vi "RemoteVI Complex Fixture.vi"() -> ()   [LabVIEW 2020]
doc: "This example demonstrates the use of splitter bars to divide the front panel into multiple panes. Each pane can be set up to behave differently depending on the desired function of each pane. In this example the graphical display contained in the lower right pane has the ability to resize with the pane."
uses:
  source/RemoteVI.lvlib
panel:
  in  "Nav":string(tree)="tag_item1"
  out "error out":errorcluster
  in  "Inspector":bool
  in  "Stop":bool
  in  "Steps":cluster{"Name":string, "Value":dbl, "On":bool}[](array[cluster])
  in  "Results":string[][](table)
  in  "Log Path":path
  out "Status":string
  in  "View":i32(ring) items=["View A", "View B"]
  in  "Settings":enum32{"Acquisition", "Display", "Viewer"}(tab)
  in  "Channel":T1
  in  "Rate":dbl(slide)=154517.79084245834 scale=1.0..205410.22592152198 scale format="%#_6p"
  in  "Level":dbl(knob)=22413.793103448275 scale=1.0..100000.0 scale format="%#_6p"
  in  "Data File":path
  out "Scope":dbl[][](graph)
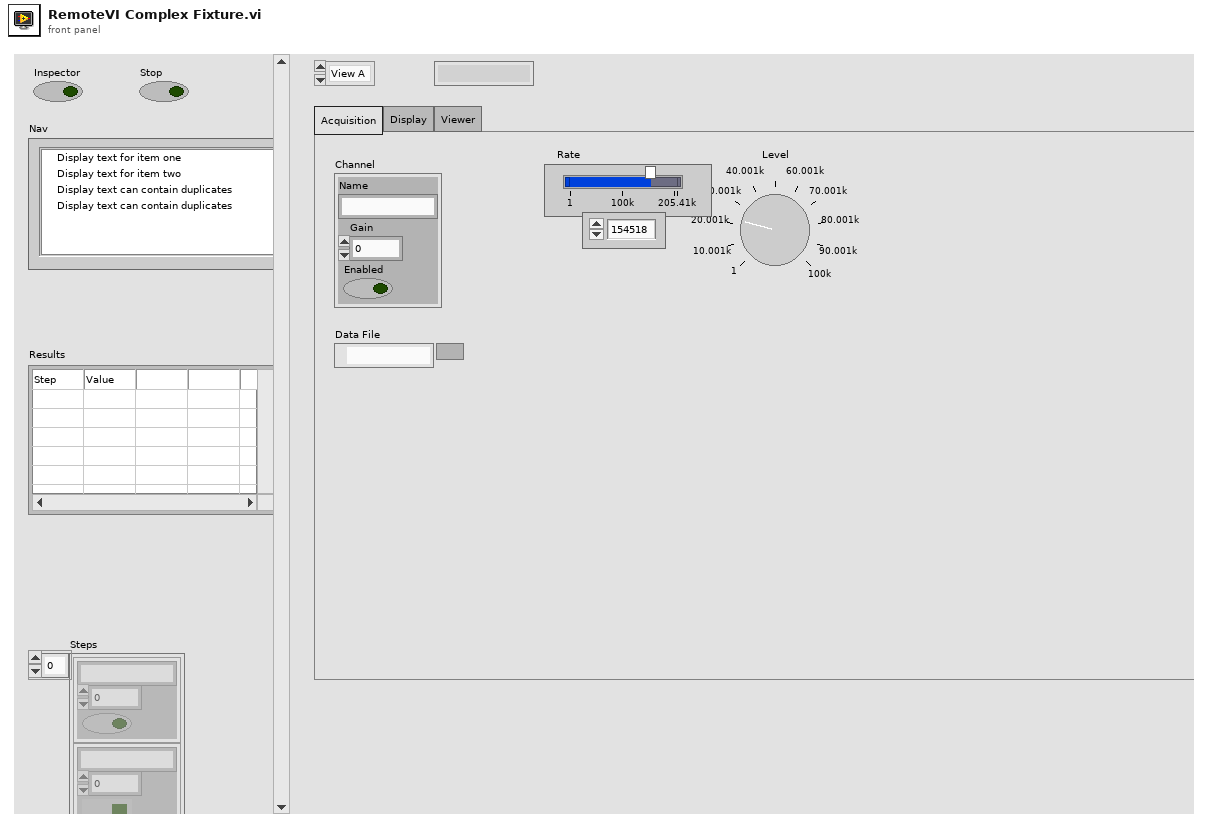
[diagram p1: front panel]
types:
  T1 = cluster{"Name":string, "Gain":dbl, "Enabled":bool}
  T2 = enum16{"open", "replace", "create", "open or create", "replace or create", "replace or create with confirmation"}
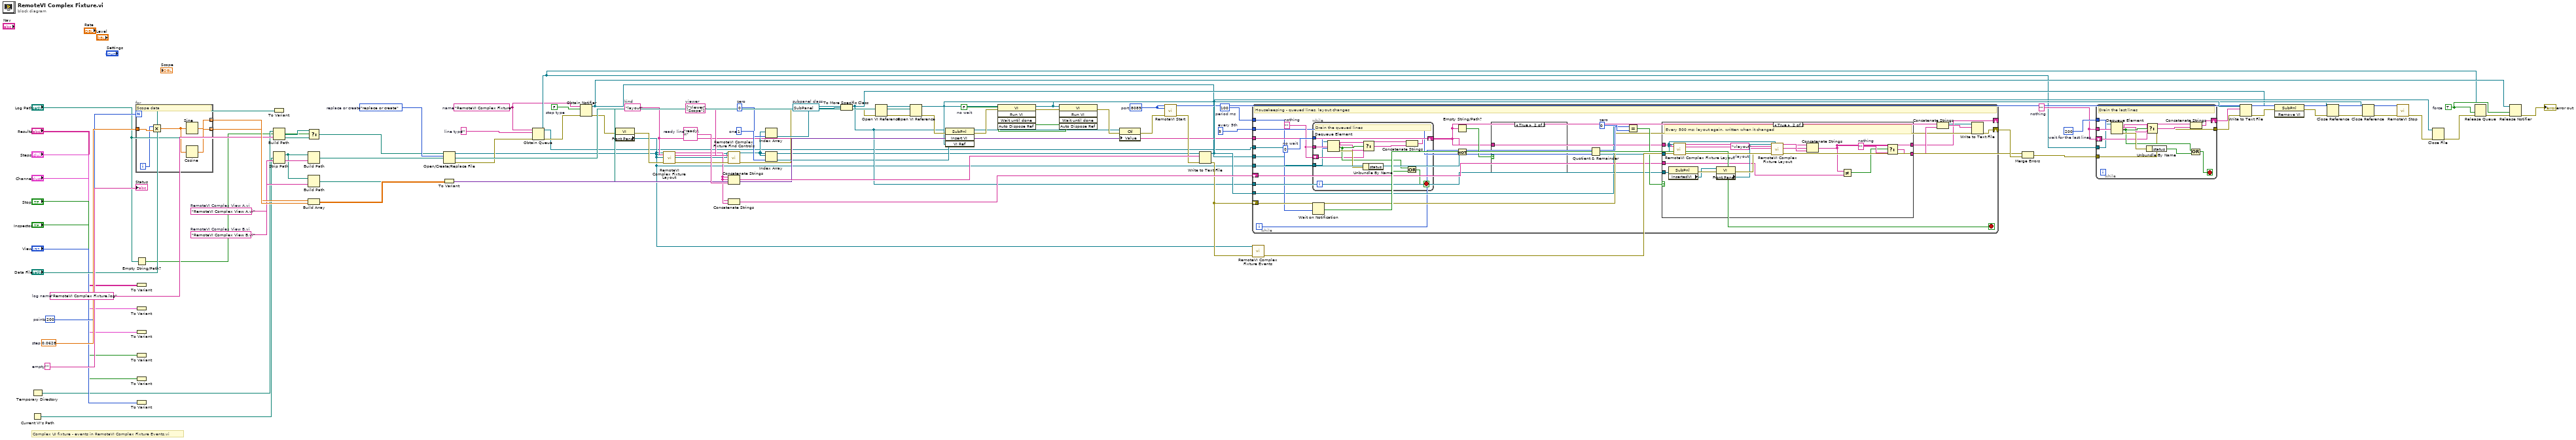
[diagram p0: block diagram]
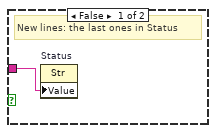
[diagram p2: hidden frame]
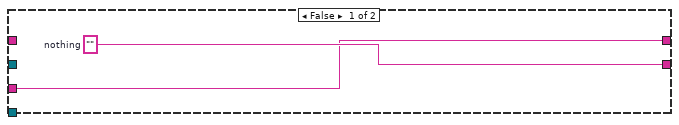
[diagram p3: hidden frame]
diagram:
  w84 = TRUE  # force
  w75 = 200  # wait for the last lines
  w74 = ""  # nothing
  w72 = ""  # empty
  w70 = 5  # every 5th
  w69 = 100  # period ms
  w63 = "ready\n"  # ready line
  w61 = u16 8089  # port
  w55 = 0.0628  # step
  w54 = 200  # points
  w51 = FALSE  # no wait
  w44 = "RemoteVI Complex View B.vi"  # RemoteVI Complex View B.vi
  w42 = "RemoteVI Complex View A.vi"  # RemoteVI Complex View A.vi
  w37 = refnum<vi> refnum  # subpanel class
  w34 = 1  # one
  w33 = 0  # zero
  w30 = string[] ["Viewer", "Scope"]  # viewer
  w19 = "layout"  # kind
  w12 = FALSE  # stop type
  w11 = ""  # line type
  w10 = "RemoteVI Complex Fixture"  # name
  w7 = T2."replace or create"  # replace or create
  w4 = "RemoteVI Complex Fixture.log"  # log name
  # "Complex UI fixture - events in RemoteVI Complex Fixture Events.vi"
  n1 = Temporary Directory() -> (w3:path)
  n2 = Current VI's Path() -> (path=w40:path)
  n3 = for {
    N: w54 -> [_]
    tunnel: w55 -> [w88]
    tunnel: [w90] -> w56 mode=indexing
    tunnel: [w91] -> w57 mode=indexing
    i -> [w87]
    # "Scope data"
    n4 = Multiply(x=w87, y=w88) -> (x*y=w89:dbl)
    n5 = Sine(x=w89) -> (sin(x)=w90:dbl)
    n6 = Cosine(x=w89) -> (cos(x)=w91:dbl)
  }
  n7 = Empty String/Path?(string/path="Log Path") -> (empty?=w2:bool)
  n8 = To Variant(anything="Results") -> ()  [unwired: 1 out]
  n9 = To Variant(anything="Steps") -> ()  [unwired: 1 out]
  n10 = To Variant(anything="Channel") -> ()  [unwired: 1 out]
  n11 = To Variant(anything="Stop") -> ()  [unwired: 1 out]
  n12 = To Variant(anything="Inspector") -> ()  [unwired: 1 out]
  n13 = To Variant(anything="View") -> ()  [unwired: 1 out]
  n14 = To Variant(anything="Data File") -> ()  [unwired: 1 out]
  n15 = Build Path(base path=w3, name or relative path=w4) -> (appended path=w5:path)
  n16 = Strip Path(path=w40) -> (stripped path=w41:path)  [unwired: 1 out]
  n17 = Select(t=w5, s=w2, f="Log Path") -> (s? t:f=w6:path)
  n18 = Build Path(base path=w41, name or relative path=w42) -> (appended path=w43:path)
  n19 = Build Path(base path=w41, name or relative path=w44) -> (appended path=w45:path)
  n20 = Build Array(w56, w57) -> (w58:dbl[][])
  n21 = Open/Create/Replace File(file path (use dialog)=w6, operation (0:open)=w7) -> (refnum out=w8:refnum<file>, error out=w9:errorcluster)  [unwired: 4 in, 1 out]
  n22 = To Variant(anything=w58) -> (Variant=w59:variant)
  n23 = Obtain Queue(name (unnamed)=w10, element data type=w11, error in (no error)=w9) -> (queue out=w13:refnum<queue>, error out=w14:errorcluster)  [unwired: 2 in, 1 out]
  n24 = Obtain Notifier(name (unnamed)=w10, notification data type=w12, error in (no error)=w14) -> (notifier out=w15:refnum<notifier>, error out=w16:errorcluster)  [unwired: 1 in, 1 out]
  n25 = property class="VI"(error in=w16) -> (error out=w18:errorcluster, "Front Panel"=w17:refnum<vi>)  [unwired: 1 in, 1 out]
  n26 = call "RemoteVI Complex Fixture Layout.vi"("Panel"=w17, "kind"=w19, "Host Panel"=w17, "error in"=w18) -> ("layout"=w20:string, "panes"=w21:string, "error out"=w22:errorcluster)  [unwired: 9 in]
  n27 = call "RemoteVI Complex Fixture Find Controls.vi"("Panel"=w17, "labels"=w30, "error in"=w22) -> ("Controls"=w31:refnum<vi>[], "error out"=w32:errorcluster)  [unwired: 11 in]
  n28 = Concatenate Strings(w20, w21, w63) -> (w64:string)
  n29 = Concatenate Strings(w20, w21) -> (w67:string)
  n30 = Index Array(array=w31, index=w33) -> (element=w35:refnum<vi>)
  n31 = Index Array(array=w31, index=w34) -> (element=w36:refnum<vi>)
  n32 = To More Specific Class(target class=w37, reference=w35, error in=w32) -> (specific class reference=w38:refnum<vi>, error out=w39:errorcluster)
  n33 = Open VI Reference(vi path=w43, error in (no error)=w39) -> (vi reference=w46:refnum<vi>, error out=w47:errorcluster)  [unwired: 4 in]
  n34 = Open VI Reference(vi path=w45, error in (no error)=w47) -> (vi reference=w48:refnum<vi>, error out=w49:errorcluster)  [unwired: 4 in]
  n35 = invoke class="SubPnl" method="Insert VI"(reference=w38, error in=w49, "VI Ref"=w46) -> (error out=w50:errorcluster)  [unwired: 1 in, 3 out]
  n36 = invoke class="VI" method="Run VI"(reference=w46, error in=w50, "Wait until done"=w51, "Auto Dispose Ref"=w51) -> (error out=w52:errorcluster)  [unwired: 1 in, 4 out]
  n37 = invoke class="VI" method="Run VI"(reference=w48, error in=w52, "Wait until done"=w51, "Auto Dispose Ref"=w51) -> (error out=w53:errorcluster)  [unwired: 1 in, 4 out]
  n38 = property class="Ctl"(reference=w36, error in=w53, "Value"=w59) -> (error out=w60:errorcluster)  [unwired: 1 out]
  n39 = call "RemoteVI Start.vi"("port"=w61, "error in"=w60) -> ("error out"=w62:errorcluster)  [unwired: 12 in, 1 out]
  n40 = Write to Text File(file (use dialog)=w8, text=w64, error in=w62) -> (refnum out=w65:refnum<file>, error out=w66:errorcluster)  [unwired: 1 in, 1 out]
  n41 = while {
    tunnel: w69 -> [w96]
    tunnel: w70 -> [w98]
    tunnel: w19 -> [w99]
    tunnel: w13 -> [w94]
    tunnel: w15 -> [w93]
    tunnel: w17 -> [w97]
    shift-right: [w102] -> _
    shift-left: w67 -> [w101]
    tunnel: w38 -> [w100]
    tunnel: w65 -> [w95]
    shift-right: [w104] -> w71
    shift-left: w66 -> [w103]
    i -> [w92]
    stop <- w115 stop-if-true
    w110 = 0  # zero
    w107 = 0  # no wait
    w106 = ""  # nothing
    # "Housekeeping - queued lines, layout changes"
    n42 = while {
      tunnel: w107 -> [w136]
      tunnel: w106 -> [w137]
      shift-right: [w139] -> w108
      shift-left: w106 -> [w138]
      tunnel: w94 -> [w135]
      stop <- w145 stop-if-true
      # "Drain the queued lines"
      n43 = Dequeue Element(queue=w135, timeout in ms (-1)=w136) -> (element=w140:string, timed out?=w141:bool, error out=w142:errorcluster)  [unwired: 1 in, 1 out]
      n44 = Select(t=w137, s=w141, f=w140) -> (s? t:f=w143:string)
      n45 = Unbundle By Name(w142) -> ("status"=w144:bool)
      n46 = Concatenate Strings(w138, w143) -> (w139:string)
      n47 = Or(x=w141, y=w144) -> (x .or. y?=w145:bool)
    }
    n48 = Wait on Notification(notifier=w93, timeout in ms (-1)=w96) -> (timed out?=w105:bool)  [unwired: 2 in, 3 out]
    n49 = Empty String/Path?(string/path=w108) -> (empty?=w114:bool)
    n50 = Not(x=w105) -> (.not. x?=w115:bool)
    n51 = case shown="True" w114 {
      tunnel: w108 -> [w116 _]
      frame False {
        # "New lines: the last ones in Status"
        n52 = property on="Status" class="Str"("Value"=w116) -> ()  [unwired: 2 in, 2 out]
      }
      frame True {
      }
    }
    n53 = Quotient & Remainder(x=w92, y=w98) -> (x-y*floor(x/y)=w109:i32)  [unwired: 1 out]
    n54 = Equal?(x=w109, y=w110) -> (x = y?=w111:bool)
    n55 = case shown="True" w111 {
      tunnel: w99 -> [_ w121]
      tunnel: w97 -> [_ w119]
      tunnel: w101 -> [w117 w120]
      tunnel: w100 -> [_ w122]
      tunnel: [w117 w131] -> w102
      tunnel: [w118 w134] -> w112
      frame False {
        w118 = ""  # nothing
      }
      frame True {
        w133 = ""  # nothing
        w129 = "vlayout"  # vlayout
        # "Every 500 ms: layout again, written when it changed"
        n56 = property class="SubPnl"(reference=w122) -> (error out=w126:errorcluster, "InsertedVI"=w125:refnum<vi>)  [unwired: 1 in, 1 out]
        n57 = call "RemoteVI Complex Fixture Layout.vi"("Panel"=w119, "kind"=w121, "Host Panel"=w119) -> ("layout"=w123:string, "panes"=w124:string)  [unwired: 10 in, 1 out]
        n58 = property class="VI"(reference=w125, error in=w126) -> (error out=w128:errorcluster, "Front Panel"=w127:refnum<vi>)  [unwired: 1 out]
        n59 = call "RemoteVI Complex Fixture Layout.vi"("Panel"=w127, "kind"=w129, "Host Panel"=w119, "error in"=w128) -> ("layout"=w130:string)  [unwired: 9 in, 2 out]
        n60 = Concatenate Strings(w123, w124, w130) -> (w131:string)
        n61 = Not Equal?(x=w131, y=w120) -> (x != y?=w132:bool)
        n62 = Select(t=w131, s=w132, f=w133) -> (s? t:f=w134:string)
      }
    }
    n63 = Concatenate Strings(w108, w112) -> (w113:string)
    n64 = Write to Text File(file (use dialog)=w95, text=w113, error in=w103) -> (error out=w104:errorcluster)  [unwired: 1 in, 2 out]
  }
  n65 = call "RemoteVI Complex Fixture Events.vi"("Panel"=w17, "error in"=w66) -> ("error out"=w68:errorcluster)  [unwired: 13 in]
  n66 = Merge Errors(w68, w71) -> (w73:errorcluster)
  n67 = while {
    tunnel: w75 -> [w147]
    tunnel: w74 -> [w148]
    shift-right: [w151] -> w76
    shift-left: w74 -> [w150]
    tunnel: w13 -> [w146]
    tunnel: w73 -> [w149]
    tunnel: [w149] -> w77
    stop <- w157 stop-if-true
    # "Drain the last lines"
    n68 = Dequeue Element(queue=w146, timeout in ms (-1)=w147) -> (element=w152:string, timed out?=w153:bool, error out=w154:errorcluster)  [unwired: 1 in, 1 out]
    n69 = Select(t=w148, s=w153, f=w152) -> (s? t:f=w155:string)
    n70 = Unbundle By Name(w154) -> ("status"=w156:bool)
    n71 = Concatenate Strings(w150, w155) -> (w151:string)
    n72 = Or(x=w153, y=w156) -> (x .or. y?=w157:bool)
  }
  n73 = Write to Text File(file (use dialog)=w65, text=w76, error in=w77) -> (error out=w78:errorcluster)  [unwired: 1 in, 2 out]
  n74 = invoke class="SubPnl" method="Remove VI"(reference=w38, error in=w78) -> (error out=w79:errorcluster)  [unwired: 1 in, 2 out]
  n75 = Close Reference(reference=w46, error in (no error)=w79) -> (error out=w80:errorcluster)
  n76 = Close Reference(reference=w48, error in (no error)=w80) -> (error out=w81:errorcluster)
  n77 = call "RemoteVI Stop.vi"("port"=w61, "error in"=w81) -> ("error out"=w82:errorcluster)  [unwired: 13 in]
  n78 = Close File(refnum=w65, error in=w82) -> (error out=w83:errorcluster)  [unwired: 1 out]
  n79 = Release Queue(queue=w13, force destroy? (F)=w84, error in (no error)=w83) -> (error out=w85:errorcluster)  [unwired: 2 out]
  n80 = Release Notifier(notifier=w15, force destroy? (F)=w84, error in (no error)=w85) -> (error out=→"error out":errorcluster)  [unwired: 2 out]
  "Status" <- w72
